vi "Trajectory_SampleReverse.vi"(9 "Time":dbl, 11 "InputTRAJECTORY":T5 {"States"."POSE"."ROTATION"."SIN" format="%13.4f"; "States"."POSE"."ROTATION"."COS" format="%13.4f"; "States"."POSE"."ROTATION"."VALUE" format="%13.4f"; "States"."POSE"."TRANSLATION"."Y" format="%14.3f"; "States"."POSE"."TRANSLATION"."X" format="%14.3f"; "TotalTImeSecs" format="%20.3f"}) -> (3 "OutputTRAJ_STATE":T1={"TimeSeconds"=0.0, "Velocity"=0.0, "Acceleration"=0.0, "POSE"={"TRANSLATION"={"X"=0.0, "Y"=0.0}, "ROTATION"={"VALUE"=0.0, "COS"=1.0, "SIN"=0.0}}, "Curvature"=0.0} {"POSE"."ROTATION"."SIN" format="%13.4f"; "POSE"."ROTATION"."COS" format="%13.4f"; "POSE"."ROTATION"."VALUE" format="%13.4f"; "POSE"."TRANSLATION"."Y" format="%14.3f"; "POSE"."TRANSLATION"."X" format="%14.3f"})   [LabVIEW 2019, in "Trajectory_Library.lvlib"]
doc: "Sample the trajectory at a point in time. The trajectory is sampled in reverse such that the ending time becomes 0 and the beginning time is the maximum time. The selected trajectory state is then transformed to be relative to end of the trajectory.\n\nFor this subVI to work correctly, sampling must start at time 0.0. \n\nThe result is a relative trajectory which starts at 0,0,0. This assumes that the robot follows the trajectory such that the orientation of the robot equals the ending state of the trajectory. \n\nThis routine does not exist in WPILIB\n \nParameters:\n - InputTrajectory - The Trajectory data structure\n - time - The point in time since the beginning of the trajectory to sample. (seconds)\n\nReturns:\n - OutputTrajState - The state at that point in time."
uses:
  Trajectory_Library.lvlib
  TypeDef/TRANSLATION2D.ctl
  TypeDef/ROTATION2D.ctl
  TypeDef/POSE2D.ctl
  TypeDef/TRAJ_STATE.ctl
  TypeDef/TRAJECTORY.ctl
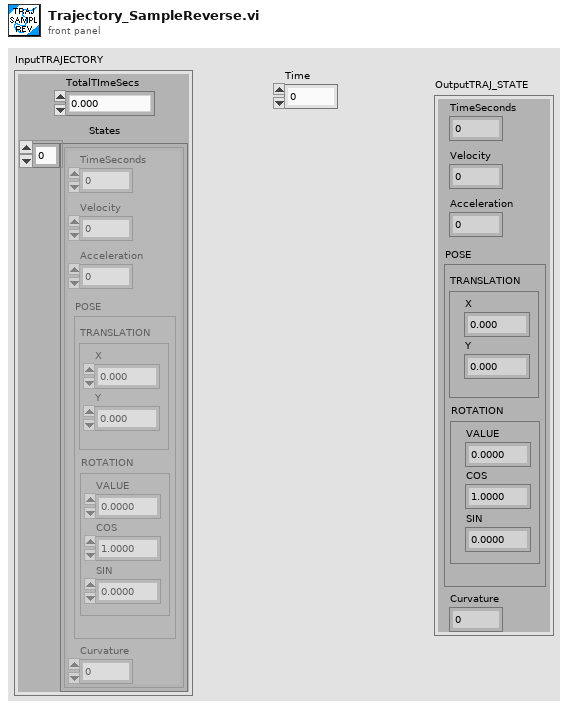
[diagram p1: front panel]
types:
  T1 = typedef "Trajectory_Library.lvlib/TRAJ_STATE.ctl" = cluster{"TimeSeconds":dbl, "Velocity":dbl, "Acceleration":dbl, "POSE":T2, "Curvature":dbl}
  T2 = typedef "Trajectory_Library.lvlib/POSE2D.ctl" = cluster{"TRANSLATION":T3, "ROTATION":T4}
  T3 = typedef "Trajectory_Library.lvlib/TRANSLATION2D.ctl" = cluster{"X":dbl, "Y":dbl}
  T4 = typedef "Trajectory_Library.lvlib/ROTATION2D.ctl" = cluster{"VALUE":dbl, "COS":dbl, "SIN":dbl}
  T5 = typedef "Trajectory_Library.lvlib/TRAJECTORY.ctl" = cluster{"TotalTImeSecs":dbl, "States":T1[]}
  T6 = typedef "WPILib_Math.lvlib/TRANSFORM2D.ctl" = cluster{"TRANSLATION":T7, "ROTATION":T8, "xF":bool}
  T7 = typedef "WPILib_Math.lvlib/TRANSLATION2D.ctl" = cluster{"X":dbl, "Y":dbl}
  T8 = typedef "WPILib_Math.lvlib/ROTATION2D.ctl" = cluster{"VALUE":dbl, "COS":dbl, "SIN":dbl}
  T9 = typedef "WPILib_Math.lvlib/POSE2D.ctl" = cluster{"TRANSLATION":T7, "ROTATION":T8}
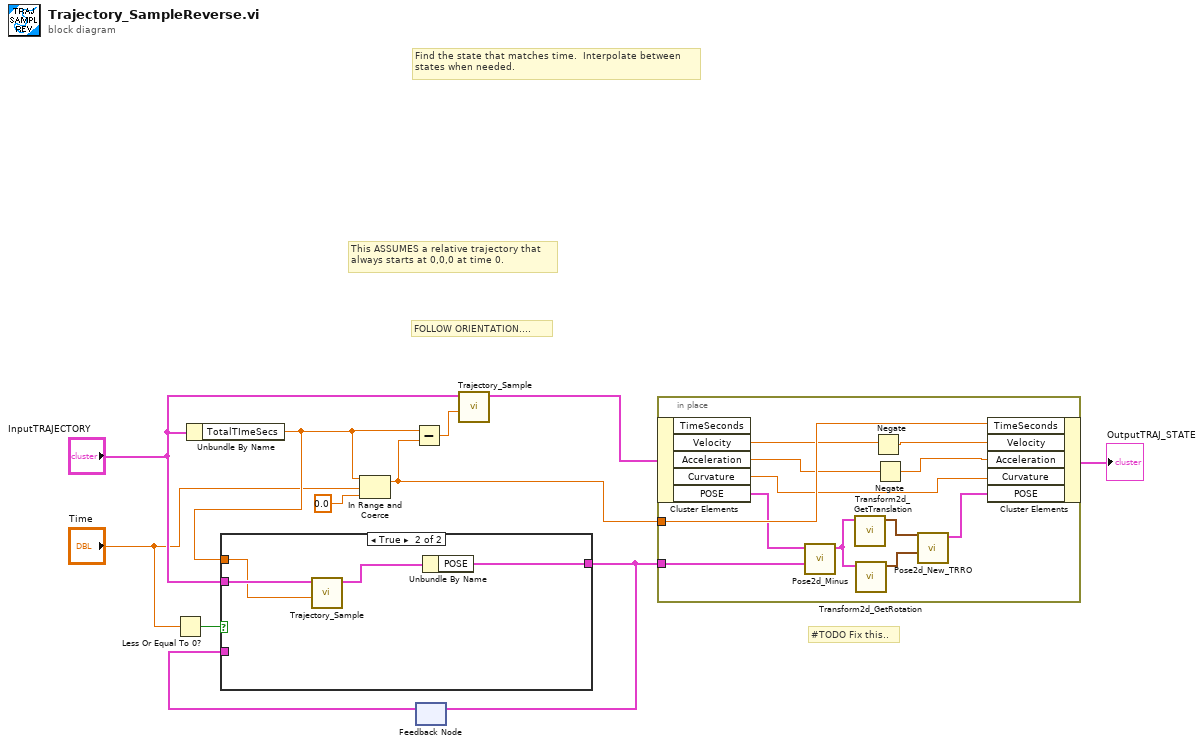
[diagram p0: block diagram]
diagram:
  # "#TODO Fix this.."
  # "This ASSUMES a relative trajectory that \nalways starts at 0,0,0 at time 0."
  # "FOLLOW ORIENTATION...."
  # "Find the state that matches time.  Interpolate between\nstates when needed."
  n1 = Less Or Equal To 0?(x="Time") -> (x <= 0?=w11:bool)
  n2 = Unbundle By Name("InputTRAJECTORY") -> ("TotalTImeSecs"=w6:dbl)
  n3 = In Range and Coerce(upper limit=w6, x="Time", lower limit=0.0) -> (coerced(x)=w5:dbl)  [unwired: 1 out]
  n4 = Subtract(x=w6, y=w5) -> (x-y=w4:dbl)
  n5 = feedback #1() -> (w9:T2)  [unwired: 1 in]
  n6 = case shown="True" w11 {
    tunnel: "InputTRAJECTORY" -> [_ w15]
    tunnel: w6 -> [_ w14]
    tunnel: [w12 w13] -> w8
    tunnel: w9 -> [w12 _]
    frame False {
    }
    frame True {
      n7 = call "Trajectory_Sample.vi"("Time"=w14, "InputTRAJECTORY"=w15) -> ("OutputTRAJ_STATE"=w16:T1)  [unwired: 9 in]
      n8 = Unbundle By Name(w16) -> ("POSE"=w13:T2)
    }
  }
  n9 = feedback-in #1(w8) -> ()
  n10 = call "Trajectory_Sample.vi"("Time"=w4, "InputTRAJECTORY"="InputTRAJECTORY") -> ("OutputTRAJ_STATE"=w10:T1)  [unwired: 9 in]
  n11 = in-place {
    in-place-border: w5 -> [w27]
    in-place-border: w8 -> [w21]
    n12 = in-place-cluster #2(w10) -> ("Velocity"=w26:dbl, "Acceleration"=w24:dbl, "Curvature"=w23:dbl, "POSE"=w22:T2)  [unwired: 1 out]
    n13 = call "Pose2d_Minus.vi"("other POSE"=w21, "in POSE"=w22) -> ("outTRANSFORM"=w20:T6)  [unwired: 9 in]
    n14 = call "Transform2d_GetTranslation.vi"("inTRANSFORM"=w20) -> ("TRANSLATION"=w19:T7)  [unwired: 10 in]
    n15 = call "Transform2d_GetRotation.vi"("inTRANSFORM"=w20) -> ("ROTATION"=w18:T8)  [unwired: 10 in]
    n16 = Negate(x=w26) -> (-x=w25:dbl)
    n17 = Negate(x=w24) -> ()  [unwired: 1 out]
    n18 = call "Pose2d_New_TRRO.vi"("ROTATION"=w18, "TRANSLATION"=w19) -> ("outPOSE"=w17:T9)  [unwired: 9 in]
    n19 = in-place-cluster #2("TimeSeconds"=w27, "Velocity"=w25, "Acceleration"=w24, "Curvature"=w23, "POSE"=w17) -> (→"OutputTRAJ_STATE":T1)
  }
